vi "AdaptToInputs.vi"(0 "XRef":T10, 1 "Term Types":T7, 2 "State In":T1) -> (14 "Reply":T5, 15 "Fatal Error Out":T4, 16 "State Out":T1)   [LabVIEW 2021, in "FirstXNode .xnode"]
uses:
  FirstXNode .xnode
  <vilib>/XNodeSupport/XNodeXNodeRef.ctl
  <vilib>/XNodeSupport/XNodeTermTypeIDPairs.ctl
  <vilib>/XNodeSupport/XNodeTermTypeIDPair.ctl
  <vilib>/XNodeSupport/XNodeType.ctl
  <vilib>/XNodeSupport/XNodeString.ctl
  State.ctl
  <vilib>/XNodeSupport/XNodeBounds.ctl
  <vilib>/XNodeSupport/XNodeInt.ctl
  <vilib>/XNodeSupport/XNodeStringArray.ctl
  <vilib>/XNodeSupport/XNodeErrorCluster.ctl
  <vilib>/Utility/Data Type/Type Definitions/Data Type.ctl
  <vilib>/XNodeSupport/NI_XNodeSupport.lvlib
  <vilib>/Utility/Data Type/NI_Data Type.lvlib
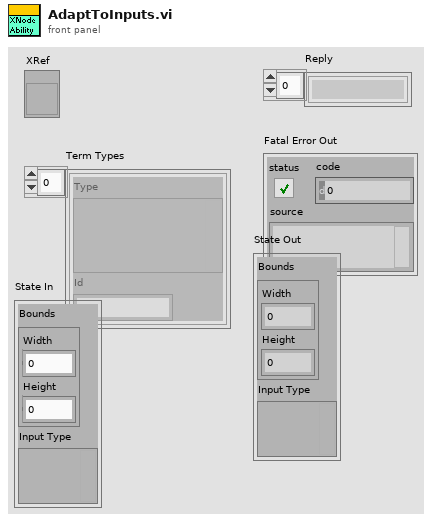
[diagram p1: front panel]
types:
  T1 = typedef "FirstXNode .xnode/State.ctl" = cluster{"Bounds":T2, "Input Type":variant}
  T2 = typedef "NI_XNodeSupport.lvlib/XNodeBounds.ctl" = cluster{"Width":T3, "Height":T3}
  T3 = typedef "NI_XNodeSupport.lvlib/XNodeInt.ctl" = i32
  T4 = typedef "NI_XNodeSupport.lvlib/XNodeErrorCluster.ctl" = errorcluster
  T5 = typedef "NI_XNodeSupport.lvlib/XNodeStringArray.ctl" = T6[]
  T6 = typedef "NI_XNodeSupport.lvlib/XNodeString.ctl" = string
  T7 = typedef "NI_XNodeSupport.lvlib/XNodeTermTypeIDPairs.ctl" = T8[]
  T8 = typedef "NI_XNodeSupport.lvlib/XNodeTermTypeIDPair.ctl" = cluster{"Type":T9, "Id":T6}
  T9 = typedef "NI_XNodeSupport.lvlib/XNodeType.ctl" = variant
  T10 = typedef "NI_XNodeSupport.lvlib/XNodeXNodeRef.ctl" = refnum<vi>
  T11 = typedef "NI_Data Type.lvlib/Data Type.ctl" = enum8{"Invalid Type", "Void", "I8", "I16", "I32", "I64", "U8", "U16", "U32", "U64", "Single Float", "Double Float", "Extended Float", "Single Complex", "Double Complex", "Extended Complex", "Enum U8", "Enum U16", "Enum U32", "Enum U64", "Single Float With Unit", "Double Float With Unit", "Extended Float With Unit", "Single Complex with Unit", "Double Complex with Unit", "Extended Complex with Unit", "Boolean", "String", "Path", "Picture", "Tag", "Array", "Cluster", "Variant", "LV Variant", "Waveform", "Timestamp", "Digital Waveform", "Digital Data", "ExpressData", "Refnum", "External Data", "VI", "Poly VI", "LabVIEW Class Instance", "Fixed Point", "Set Collection", "Map Collection"}
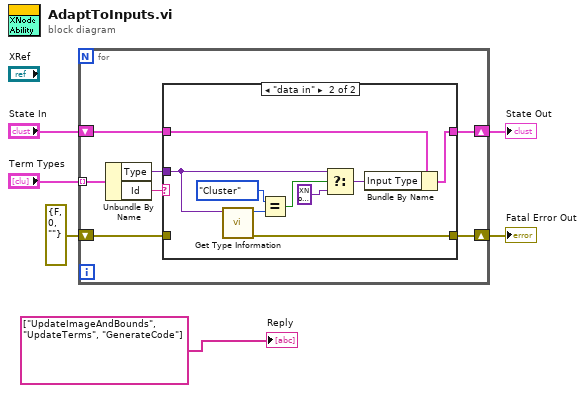
[diagram p0: block diagram]
diagram:
  n1 = for {
    tunnel: "Term Types" -> [w13] mode=indexing
    shift-right: [w9] -> w4
    shift-left: "State In" -> [w10]
    shift-right: [w8] -> w1
    shift-left: errorcluster {"status"=FALSE, "code"=0, "source"=""} ("error out") -> [w7]
    n2 = Unbundle By Name(w13) -> ("Type"=w11:T9, "Id"=w12:T6)
    n3 = case shown="\"data in\"" w12 {
      tunnel: w11 -> [_ w21]
      tunnel: w10 -> [w15 w17]
      tunnel: [w15 w16] -> w9
      tunnel: [w14 w18] -> w8
      tunnel: w7 -> [w14 _]
      frame "", Default {
      }
      frame "data in" {
        n4 = call <vilib>:"Get Type Information.vi"("variant"=w21) -> ("error out"=w18:errorcluster, "type"=w24:T11)  [unwired: 6 in, 3 out]
        n5 = Equal?(x=Data_Type."Cluster", y=w24) -> (x = y?=w22:bool)
        n6 = Select(t=w21, s=w22, f=T9 variant) -> (s? t:f=w20:T9)
        n7 = Bundle By Name(cluster=w17, "Input Type"=w20) -> (w16:T1)
      }
    }
  }
  "Fatal Error Out" <- w1
  "State Out" <- w4
  "Reply" <- T5 ["UpdateImageAndBounds", "UpdateTerms", "GenerateCode"] ("Reply")
